vi "Manual Post Build.vi"() -> ()   [LabVIEW 2019]
uses:
  <userlib>/LevyLab/Build Support/PostBuildSupport/PostBuildSupport.lvclass
panel:
  in  "Project File Path":path=path "C:/Users/patrick/Documents/GitHub/levylabpitt/Multichannel-Lockin/Multichannel Lock-In (x64).lvproj"
  out "error out":errorcluster
  in  "Output Package File Path":path=path "C:/Users/patrick/Documents/GitHub/levylabpitt/Multichannel-Lockin/builds/Package"
  in  "Product Name":string="Multichannel Lockin"
  in  "Package Version":string="2.20.0.6"
  in  "Package Source Folder":path=path "C:/Users/patrick/Documents/GitHub/levylabpitt/Multichannel-Lockin/src"
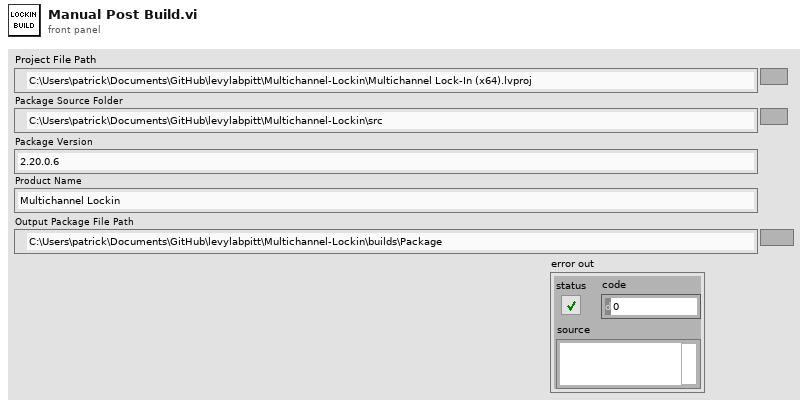
[diagram p1: front panel]
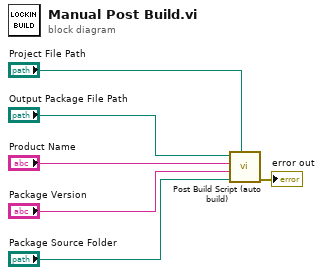
[diagram p0: block diagram]
diagram:
  n1 = call <userlib>:"Post Build Script (auto build).vi"("Project File Path"="Project File Path", "Package Source Folder"="Package Source Folder", "Package Version (Major.Minor.Fix.Build)"="Package Version", "Product Name"="Product Name", "Output Package File Path"="Output Package File Path") -> ("error out"=→"error out":errorcluster)  [unwired: 6 in]
